vi "SMTP Email [MAIL].vi"(4 "error in (no error)":errorcluster caption="entrée d'erreur (pas d'erreur)", 6 "return address":string caption="adresse de retour", 7 "smtp session":T1 caption="session smtp") -> (0 "error out":errorcluster caption="sortie d'erreur", 1 "reply":string caption="réponse", 2 "reply code":i32 caption="code de réponse", 3 "smtp session out":T1 caption="session smtp en sortie")   [LabVIEW 2022 SP3, in "Copie de NI_SMTPEmail.lvlib"]
doc: "Envoie la commande MAIL à un serveur SMTP à travers la connexion TCP décrite par \"Session SMTP\", reçoit la réponse et l'interprète. \n\nL'adresse e-mail de retour souhaitée est celle de l'utilisateur.\n\nLe VI renvoie la session SMTP en sortie et les résultats d'interprétation de l'erreur dans le cluster de sortie d'erreur."
uses:
  Copie de NI_SMTPEmail.lvlib
  SMTP Email Session.ctl
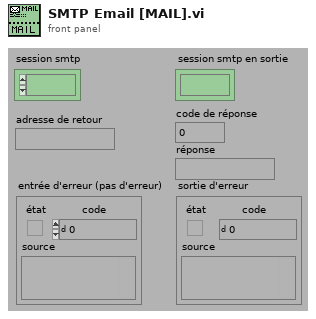
[diagram p1: front panel]
types:
  T1 = typedef "Copie de NI_SMTPEmail.lvlib/SMTP Email Session.ctl" = refnum<k1>
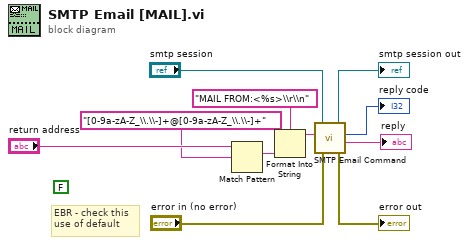
[diagram p0: block diagram]
diagram:
  (unwired) FALSE
  # "EBR - check this\nuse of default"
  n1 = Match Pattern(string="return address", regular expression="[0-9a-zA-Z_\\.\\-]+@[0-9a-zA-Z_\\.\\-]+") -> (match substring=w1:string)  [unwired: 1 in, 3 out]
  n2 = Format Into String(format string="MAIL FROM:<%s>\\r\\n", w1) -> (resulting string=w7:string)  [unwired: 2 in, 1 out]
  n3 = call "SMTP Email Command.vi"("error in (no error)"="error in (no error)", "command"=w7, "smtp session"="smtp session") -> ("error out"=→"error out":errorcluster, "reply"=→"reply":string, "reply code"=→"reply code":i32, "smtp session out"=→"smtp session out":T1)  [unwired: 1 in]
